vi "File execution not authorized--error.vi"() -> (0 "error out":errorcluster)   [LabVIEW 2026]
doc: "File execution not authorized. This means the file that should be run was not found in the corresponding whitelist."
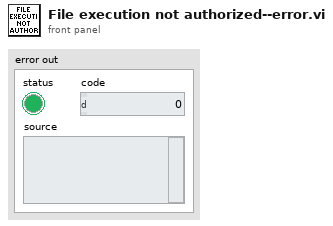
[diagram p1: front panel]
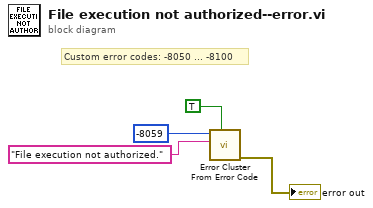
[diagram p0: block diagram]
diagram:
  # "Custom error codes: -8050 ... -8100"
  n1 = call <vilib>:"Error Cluster From Error Code.vi"("show call chain? (False)"=TRUE, "error message (\"\")"="File execution not authorized." ("error message (\"\")"), "error code (0)"=-8059) -> ("error out"=→"error out":errorcluster)  [unwired: 6 in]
